vi "ADC_Instrument_Specs.vi"(0 "Source Device":refnum<k15>="PXI1Slot2", 5 "Voltage Level Range":dbl=5.0 caption="voltage level range" format="%#.6p", 7 "Current Limit":dbl=0.1 caption="current limit" format="%#.6p", 9 "Measurement Device":enum16{"ADC"}(ring), 11 "Error In":errorcluster) -> (15 "Error Out":errorcluster)   [LabVIEW 2026, in "Core.lvlib"]
doc: "Configures the source and measurement device settings required for ADC test execution."
uses:
  Core.lvlib
  TypeDefs/Enum_Events.ctl
  TypeDefs/Enum_Event_Options.ctl
  TypeDefs/Enum_Notifier_Name.ctl
  TypeDefs/Enum_Notifier_Options.ctl
  TypeDefs/Notification_Clusters/Cluster_ADC_Instrument_Specs.ctl
panel:
  # "Instructions:\n-> Enter the configuration details for the source device\n\n-> Enter the configuration details for the measurement device"
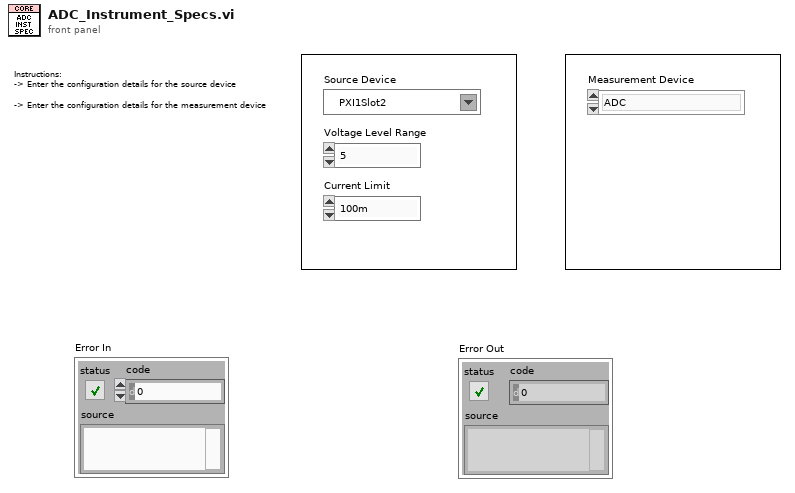
[diagram p1: front panel]
types:
  T1 = typedef "Core.lvlib/Enum_Events.ctl" = enum16{"Stop All", "Stop Subpanel", "Stop Test Spec", "Stop Result"}
  T2 = typedef "Core.lvlib/Enum_Event_Options.ctl" = enum16{"Create", "Generate", "Event Ref", "Destroy"}
  T3 = typedef "Core.lvlib/Enum_Notifier_Options.ctl" = enum16{"Create", "Send", "Status", "Release"}
  T4 = typedef "Core.lvlib/Enum_Notifier_Name.ctl" = enum16{"Device Type", "Test", "Instrument Spec", "Measurement Spec", "Status"}
  T5 = typedef "Core.lvlib/Cluster_ADC_Instrument_Specs.ctl" = cluster{"ADC Source":refnum<k15>, "Current Limit":dbl, "Voltage Level Range":dbl, "ADC DUT":string}
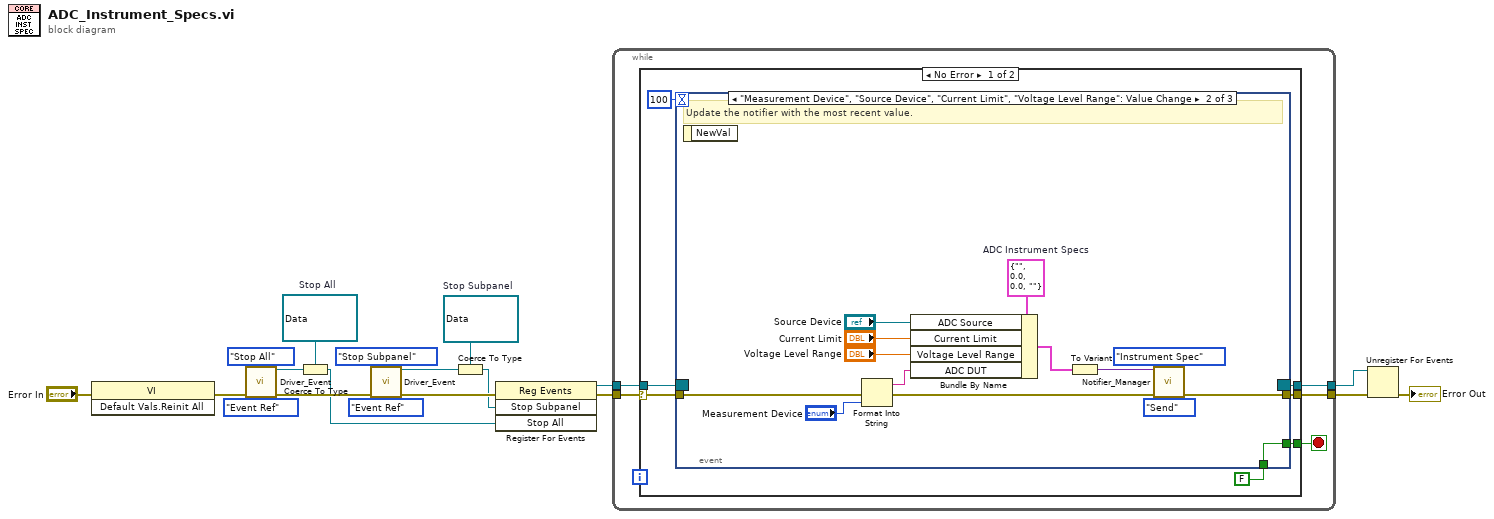
[diagram p0: block diagram]
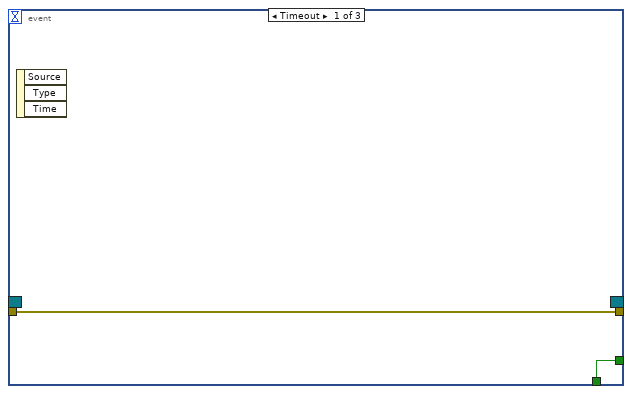
[diagram p2: hidden frame]
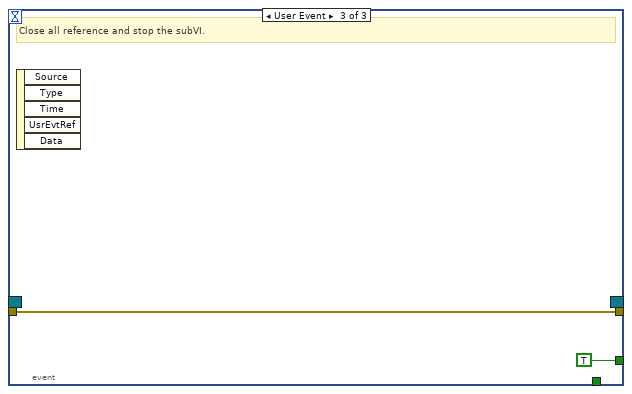
[diagram p3: hidden frame]
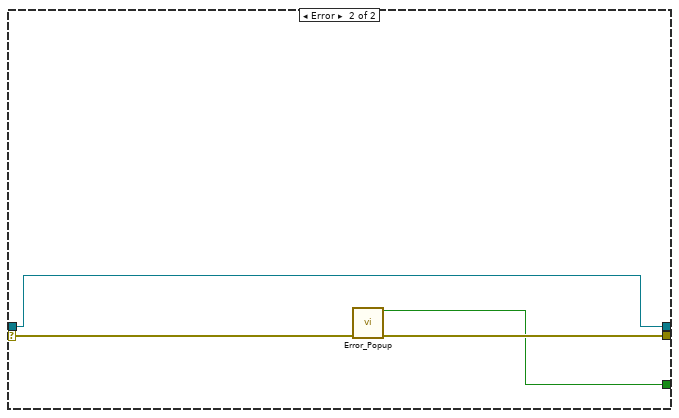
[diagram p4: hidden frame]
diagram:
  w1 = refnum<user-event> refnum  # Stop All
  w11 = refnum<user-event> refnum  # Stop Subpanel
  n1 = invoke class="VI" method="Default Vals.Reinit All"(error in="Error In") -> (error out=w7:errorcluster)  [unwired: 2 in, 2 out]
  n2 = call "Driver_Event.vi"("Event"=Enum_Events."Stop All", "Error In"=w7, "Event Operation"=Enum_Event_Options."Event Ref") -> ("Event Ref"=w3:refnum<user-event>, "Error Out"=w6:errorcluster)  [unwired: 11 in]
  n3 = Coerce To Type(0:w3, 1:w1) -> (2:w2:refnum<user-event>)
  n4 = call "Driver_Event.vi"("Event"=Enum_Events."Stop Subpanel", "Error In"=w6, "Event Operation"=Enum_Event_Options."Event Ref") -> ("Event Ref"=w18:refnum<user-event>, "Error Out"=w17:errorcluster)  [unwired: 11 in]
  n5 = Coerce To Type(0:w18, 1:w11) -> (2:w12:refnum<user-event>)
  n6 = register-events(error in=w17, w12, w2) -> (reference out=w15:refnum<event-registration>, error out=w16:errorcluster)  [unwired: 1 in]
  n7 = while {
    tunnel: w16 -> [w23]
    tunnel: [w24] -> w19
    tunnel: w15 -> [w22]
    tunnel: [w21] -> w13
    stop <- w20 stop-if-true
    n8 = case shown="No Error" w23 {
      selector: w23 -> [w30 w53]
      tunnel: [w31 w52] -> w24
      tunnel: w22 -> [w28 w51]
      tunnel: [w27 w51] -> w21
      tunnel: [w26 w50] -> w20
      frame No Error {
        n9 = event shown="[1] \"Measurement Device\", \"Source Device\", \"Current Limit\", \"Voltage Level Range\": Value Change" {
          selector: w28 -> [_ _ _]
          dyn-events: [_ _ _] -> w27
          timeout: 100 -> [_ _ _]
          tunnel: [w33 w40 w48] -> w31
          tunnel: w30 -> [w33 w41 w48]
          tunnel: [w32 w39 TRUE] -> w26
          tunnel: FALSE -> [w32 w39 _]
          event Timeout {
            n10 = event-data() -> ()  [unwired: 1 in, 3 out]
          }
          event "Measurement Device", "Source Device", "Current Limit", "Voltage Level Range": Value Change {
            w42 = T5 {"ADC Source"="", "Current Limit"=0.0, "Voltage Level Range"=0.0, "ADC DUT"=""}  # ADC Instrument Specs
            # "Update the notifier with the most recent value."
            n11 = event-data() -> ()  [unwired: 1 in, 1 out]
            n12 = Format Into String(error in=w41, "Measurement Device") -> (resulting string=w35:string, error out=w36:errorcluster)  [unwired: 2 in]
            n13 = Bundle By Name(cluster=w42, "ADC Source"="Source Device", "Current Limit"="Current Limit", "Voltage Level Range"="Voltage Level Range", "ADC DUT"=w35) -> (w44:T5)
            n14 = To Variant(anything=w44) -> (Variant=w43:variant)
            n15 = call "Notifier_Manager.vi"("Notifier Data"=w43, "Notifier Name"=Enum_Notifier_Name."Instrument Spec", "Error In"=w36, "Notifier Options"=Enum_Notifier_Options."Send") -> ("Error Out"=w40:errorcluster)  [unwired: 10 in, 1 out]
          }
          event User Event {
            # "Close all reference and stop the subVI."
            n16 = event-data() -> ()  [unwired: 1 in, 5 out]
          }
        }
      }
      frame Error {
        n17 = call "Error_Popup.vi"("Error In"=w53) -> ("Stop?"=w50:bool, "Error Out"=w52:errorcluster)  [unwired: 13 in]
      }
    }
  }
  n18 = Unregister For Events(event registration refnum=w13, error in=w19) -> (error out=→"Error Out":errorcluster)
